vi "RemoteVI Splitters Message.vi"(0 "bars":T1(array[cluster])) -> (4 "message":string)   [LabVIEW 2020, in "RemoteVI.lvlib"]
doc: "Builds the text message splitters <json> (docs\\protocol.md section 3.3) from the splitter bars RemoteVI Read Splitters.vi read: a JSON array with one object per bar, id (its index in bars), x, y, w, h (the bar in frame coordinates), vertical (true or false), min and max (the range of its left edge for a vertical bar, its top edge for a horizontal one, in frame coordinates) in that order - splitters [] when there is none. The client drags a bar itself and answers s id pos. Pure function, cannot fail. Reference: splittersMessage() in tools\\lib\\protocol.mjs, vectors tests\\vectors\\text.json (splitters)."
uses:
  RemoteVI.lvlib
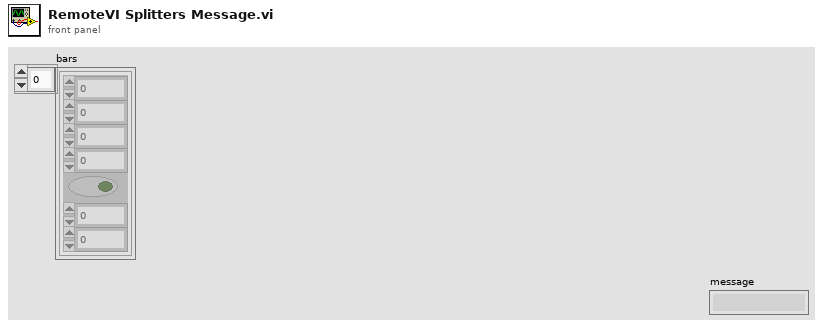
[diagram p1: front panel]
types:
  T1 = cluster{"x":i32, "y":i32, "w":i32, "h":i32, "vertical":bool, "min":i32, "max":i32}[]
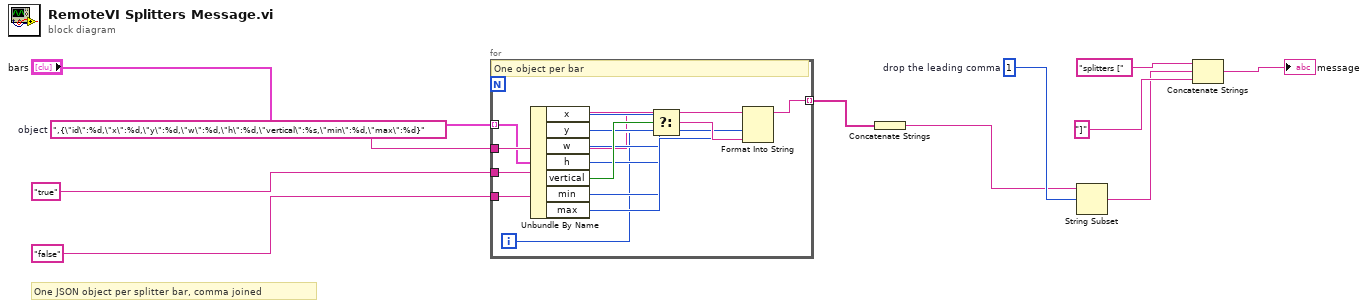
[diagram p0: block diagram]
diagram:
  w7 = 1  # drop the leading comma
  w2 = ",{\"id\":%d,\"x\":%d,\"y\":%d,\"w\":%d,\"h\":%d,\"vertical\":%s,\"min\":%d,\"max\":%d}"  # object
  # "One JSON object per splitter bar, comma joined"
  n1 = for {
    tunnel: "bars" -> [w13] mode=indexing
    tunnel: w2 -> [w14]
    tunnel: "true" -> [w15]
    tunnel: "false" -> [w16]
    tunnel: [w25] -> w5 mode=indexing
    i -> [w12]
    # "One object per bar"
    n2 = Unbundle By Name(w13) -> ("x"=w17:i32, "y"=w18:i32, "w"=w19:i32, "h"=w20:i32, "vertical"=w21:bool, "min"=w22:i32, "max"=w23:i32)
    n3 = Select(t=w15, s=w21, f=w16) -> (s? t:f=w24:string)
    n4 = Format Into String(format string=w14, w12, w17, w18, w19, w20, w24, w22, w23) -> (resulting string=w25:string)  [unwired: 2 in, 1 out]
  }
  n5 = Concatenate Strings(w5) -> (w6:string)
  n6 = String Subset(string=w6, offset (0)=w7) -> (substring=w8:string)  [unwired: 1 in]
  n7 = Concatenate Strings("splitters [", w8, "]") -> (→"message":string)
